vi "New Container.vi"(0 "Session Handle in":T2, 11 "error in (no error)":errorcluster) -> (4 "Session Handle out":T2, 6 "New Value Container":T1, 15 "error out":errorcluster)   [LabVIEW 2020, in "TSS.lvlib" / "Engine.lvclass"]
uses:
  Engine.lvclass
  Typedefs/Session Handle.ctl
  VariableContainer/Typedefs/Session Handle.ctl
  VariableContainer/VariableContainer.lvclass
  Variable Container Type.ctl
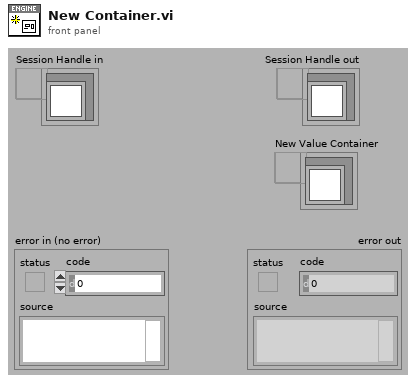
[diagram p1: front panel]
types:
  T1 = typedef "TSS.lvlib/VariableContainer.lvclass/Session Handle.ctl" = refnum<data-value>
  T2 = typedef "TSS.lvlib/Engine.lvclass/Session Handle.ctl" = refnum<data-value>
  T3 = typedef "TSS.lvlib/Engine.lvclass/Variable Container Type.ctl" = enum16{"StationGlobals", "TemporaryGlobals", "NewPropertyObject"}
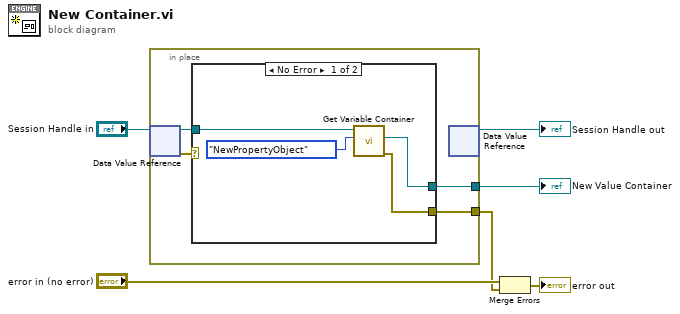
[diagram p0: block diagram]
diagram:
  n1 = in-place {
    in-place-border: [w8] -> w4
    in-place-border: [w7] -> w2
    n2 = in-place-dvr #1("Session Handle in") -> (w10:refnum<class "Engine.lvclass">, w9:errorcluster)
    n3 = case shown="No Error" w9 {
      selector: w9 -> [_ w15]
      tunnel: w10 -> [w13 _]
      tunnel: [w11 _] -> w8
      tunnel: [w12 w15] -> w7
      frame No Error {
        n4 = call "Get Variable Container.vi"("Type"=Variable_Container_Type."NewPropertyObject", "TSEngine in"=w13) -> ("error out"=w12:errorcluster, "VariableContainer"=w11:T1)  [unwired: 7 in, 1 out]
      }
      frame Error {
      }
    }
    n5 = in-place-dvr #1() -> (→"Session Handle out":T2)  [unwired: 1 in, 1 out]
  }
  "New Value Container" <- w4
  n6 = Merge Errors("error in (no error)", w2) -> (→"error out":errorcluster)
